vi "Add Packages to a Feed.vi"() -> ()   [LabVIEW 2014]
doc: "This example shows how to add packages to a feed. This example also gives the user the option of creating a new feed in the specified feed folderpath, if necessary."
uses:
  NIPM_API.lvlib
panel:
  in  "Add package":bool
  out "Package names and versions in this feed":string[][](array[string])
  in  "package (.nipkg) source filepath":path
  out "Feed created?":bool
  in  "Create new feed in folder (if necessary)":bool
  in  "feed folderpath":path
  # "1. In the Feed Information section, specify a feed folderpath and whether you want this example VI to create a new feed in the specified folder if the folder does not already contain an existing feed.\n2. In the Package to add to the feed section, set the Add package control to TRUE and browse to the filepath of the package (.nipkg) that you want to add to the feed.\n3. Run the VI.\n\nFor more information, refer to the Introduction to NIPM Feeds document on https://bit.ly/nipkg."
  # "Feed Information"
  # "Package to add to the feed"
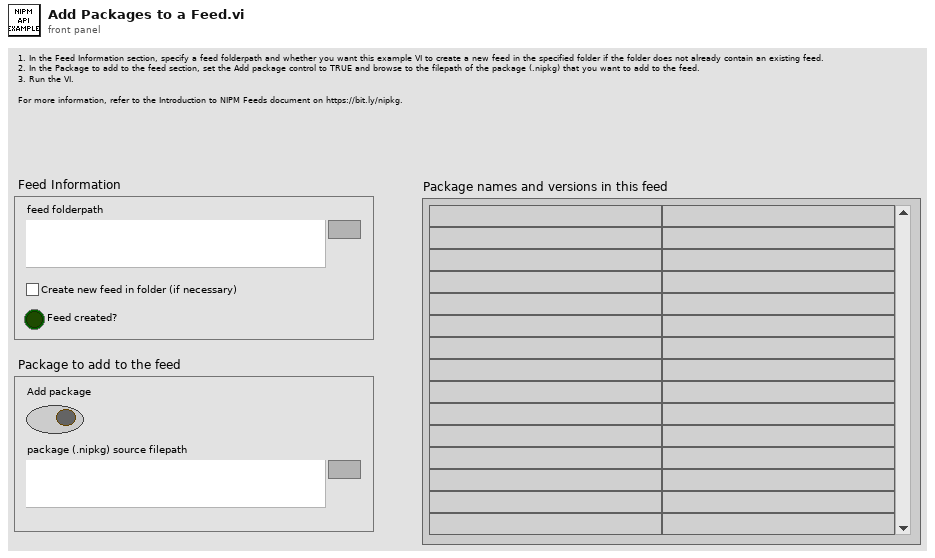
[diagram p1: front panel]
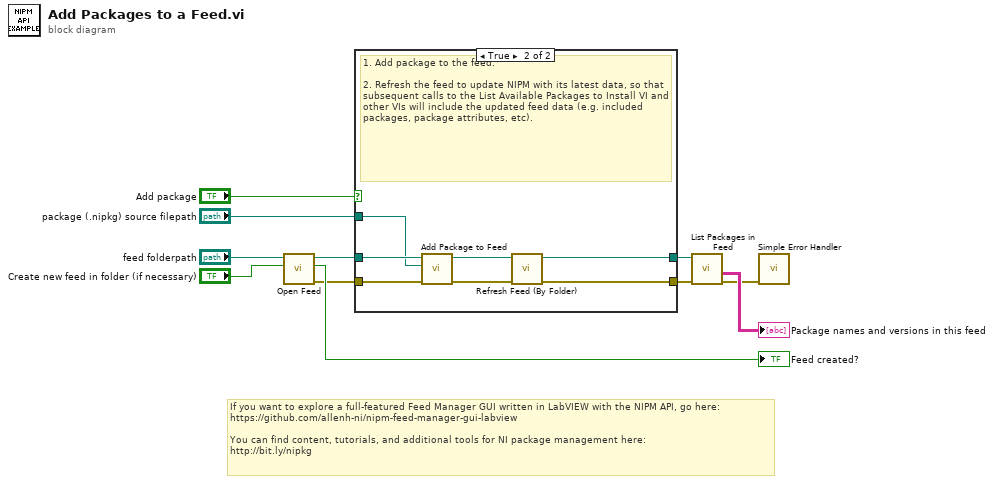
[diagram p0: block diagram]
diagram:
  # "If you want to explore a full-featured Feed Manager GUI written in LabVIEW with the NIPM API, go here:\nhttps://github.com/allenh-ni/nipm-feed-manager-gui-labview\n\nYou can find content, tutorials, and additional tools for NI package management here:\nhttp://bit.ly/nipkg"
  n1 = call "Open Feed.vi"("create feed if necessary (F)"="Create new feed in folder (if necessary)", "feed folderpath"="feed folderpath") -> ("error out"=w8:errorcluster, "feed created?"=→"Feed created?":bool, "feed folderpath out"=w5:path)  [unwired: 7 in]
  n2 = case shown="True" "Add package" {
    tunnel: w8 -> [w12 w20]
    tunnel: [w12 w14] -> w6
    tunnel: w5 -> [w13 w19]
    tunnel: [w13 w15] -> w4
    tunnel: "package (.nipkg) source filepath" -> [_ w18]
    frame False {
      # "Don't add package to the feed"
    }
    frame True {
      # "1. Add package to the feed.\n\n2. Refresh the feed to update NIPM with its latest data, so that subsequent calls to the List Available Packages to Install VI and other VIs will include the updated feed data (e.g. included packages, package attributes, etc)."
      n3 = call "Add Package to Feed.vi"("error in"=w20, "package source filepath"=w18, "feed folderpath in"=w19) -> ("error out"=w16:errorcluster, "feed folderpath out"=w17:path)  [unwired: 6 in, 1 out]
      n4 = call "Refresh Feed (By Folder).vi"("error in"=w16, "feed folderpath in"=w17) -> ("error out"=w14:errorcluster, "feed folderpath out"=w15:path)  [unwired: 8 in]
    }
  }
  n5 = call "List Packages in Feed.vi"("error in"=w6, "feed folderpath in"=w4) -> ("error out"=w2:errorcluster, "package names and versions"=→"Package names and versions in this feed":string[][])  [unwired: 6 in, 2 out]
  n6 = call <vilib>:"Simple Error Handler.vi"("error in (no error)"=w2) -> ()  [unwired: 4 in, 5 out]
